vi "eDyno AO Setup.vi"(0 "physical channels":tag, 1 "AO Range (V)":dbl=10.0, 2 "Sample Rate (S/s)":dbl=51200.0, 3 "Buffer Samples":i32=20480, 5 "error in":errorcluster) -> (14 "task out":refnum<k21>, 19 "error out":errorcluster)   [LabVIEW 2026]
doc: "Creates the AO task that plays the simulated accelerometer voltage: AO voltage channel (+/- AO Range), continuous sample clock at Sample Rate with a buffer of Buffer Samples, regeneration DISABLED (each block is new data). Not started."
uses:
  <vilib>/DAQmx/create/channels.llb/DAQmx Create Channel (AO-Voltage-Basic).vi
  <vilib>/DAQmx/configure/timing.llb/DAQmx Timing (Sample Clock).vi
  <resource>/objmgr/daqmx.rc
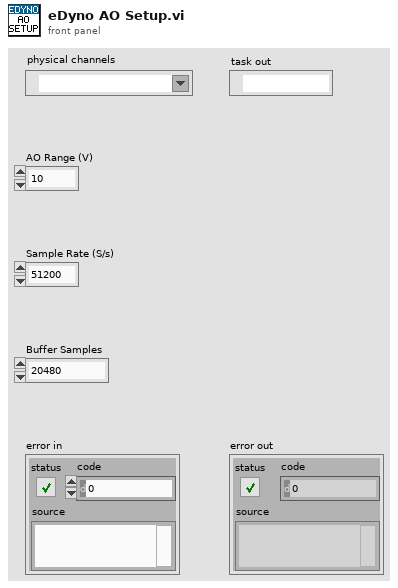
[diagram p1: front panel]
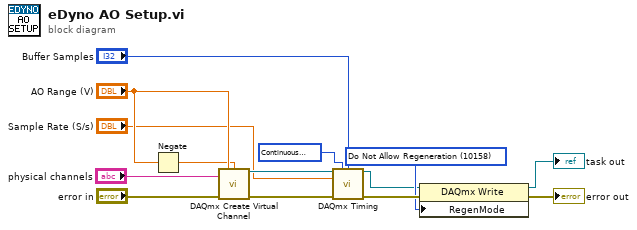
[diagram p0: block diagram]
diagram:
  w5 = 10158 items=["Allow Regeneration"=10097, "Do Not Allow Regeneration"=10158] ("RegenMode")
  w10 = 10123 items=["Finite Samples"=10178, "Continuous Samples"=10123, "Hardware Timed Single Point"=12522] ("Sample Mode")
  n1 = Negate(x="AO Range (V)") -> (-x=w13:dbl)
  n2 = call-poly <vilib>:"DAQmx Create Virtual Channel.vi"("maximum value"="AO Range (V)", "minimum value"=w13, "physical channels"="physical channels", "error in"="error in") -> ("task out"=w11:refnum<k21>, "error out"=w7:errorcluster)  [unwired: 10 in]
  n3 = call-poly <vilib>:"DAQmx Timing.vi"("task/channels in"=w11, "sample mode"=w10, "samples per channel"="Buffer Samples", "rate"="Sample Rate (S/s)", "error in"=w7) -> ("task out"=w4:refnum<k21>, "error out"=w6:errorcluster)  [unwired: 9 in]
  n4 = property class="DAQmx Write"(reference=w4, error in=w6, "RegenMode"=w5) -> (reference out=→"task out":refnum<k21>, error out=→"error out":errorcluster)
